vi "ZM-ROOT-evaluateError.vi"(8 "error in (no error)":errorcluster, 10 "stop actor? in":bool=TRUE, 11 "ZM-ROOT-root in":refnum<class "ZM-ROOT-root.lvclass">) -> (0 "error out":errorcluster, 2 "stop actor? out":bool=TRUE, 3 "ZM-ROOT-root out":refnum<class "ZM-ROOT-root.lvclass">)   [LabVIEW 2020, in "ZM-ROOT-root.lvlib" / "ZM-ROOT-root.lvclass"]
doc: "Error hook of the root, called by Handle Error and after the panel loop. For now a pass-through: the class, the error and stop actor? go out unchanged; nothing is logged or cleared. Error-handling plan: none yet; an error stops the root and, through AF's Stop Core, the whole tree."
uses:
  ZM-ROOT-root.lvclass
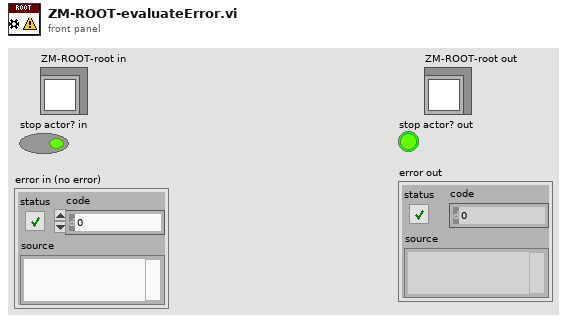
[diagram p1: front panel]
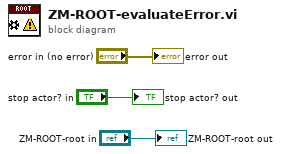
[diagram p0: block diagram]
diagram:
  "ZM-ROOT-root out" <- "ZM-ROOT-root in"
  "stop actor? out" <- "stop actor? in"
  "error out" <- "error in (no error)"
